vi "Lire un segment MODBUS EPC.vi"(0 "Port COM":refnum<visa-resource-name>, 1 "No prog":u8 caption="Numéro de programme", 2 "Adresse régulateur":u8, 3 "Numéro de segment":u8, 4 "données générales":u16[](array[numeric]), 5 "error in (no error)":errorcluster caption="entrée d'erreur (pas d'erreur)") -> (6 "Programmation Segment":T1(array[cluster]), 7 "Fin de programme":bool, 8 "error out":errorcluster caption="entrée d'erreur (pas d'erreur)")   [LabVIEW 2022 SP3]
uses:
  Variables globales/Variables glob EUROTHERM.vi
panel:
  out "Data 2 (U16)":u16[][](array[numeric])
  # "unités rampe"
  # "unités palier"
  # "nb cycles"
  # "type fin"
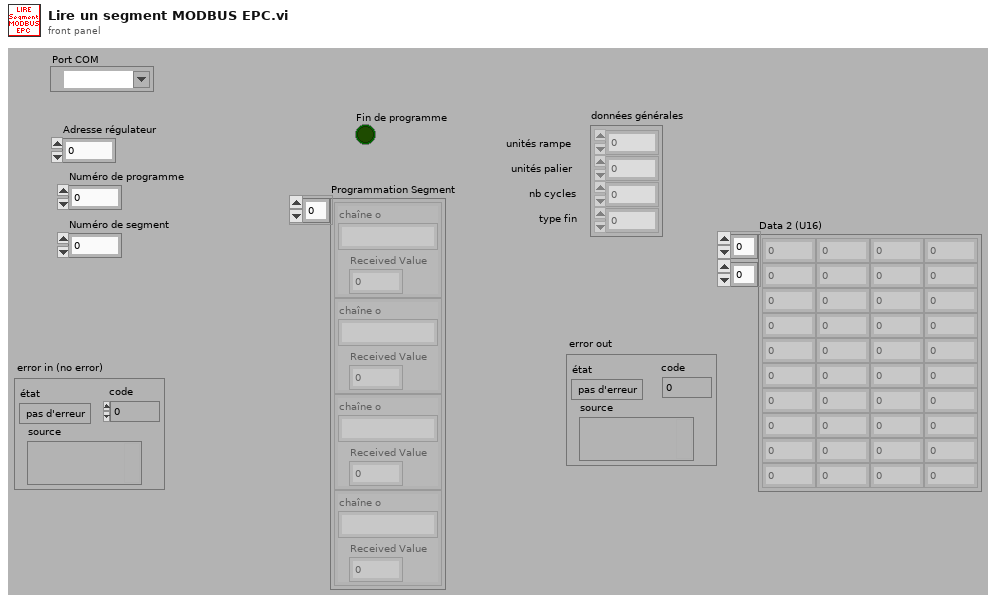
[diagram p1: front panel]
types:
  T1 = cluster{"chaîne o":string, "Received Value":dbl}[]
  T2 = typedef "Semaphore RefNum" = refnum<k1>
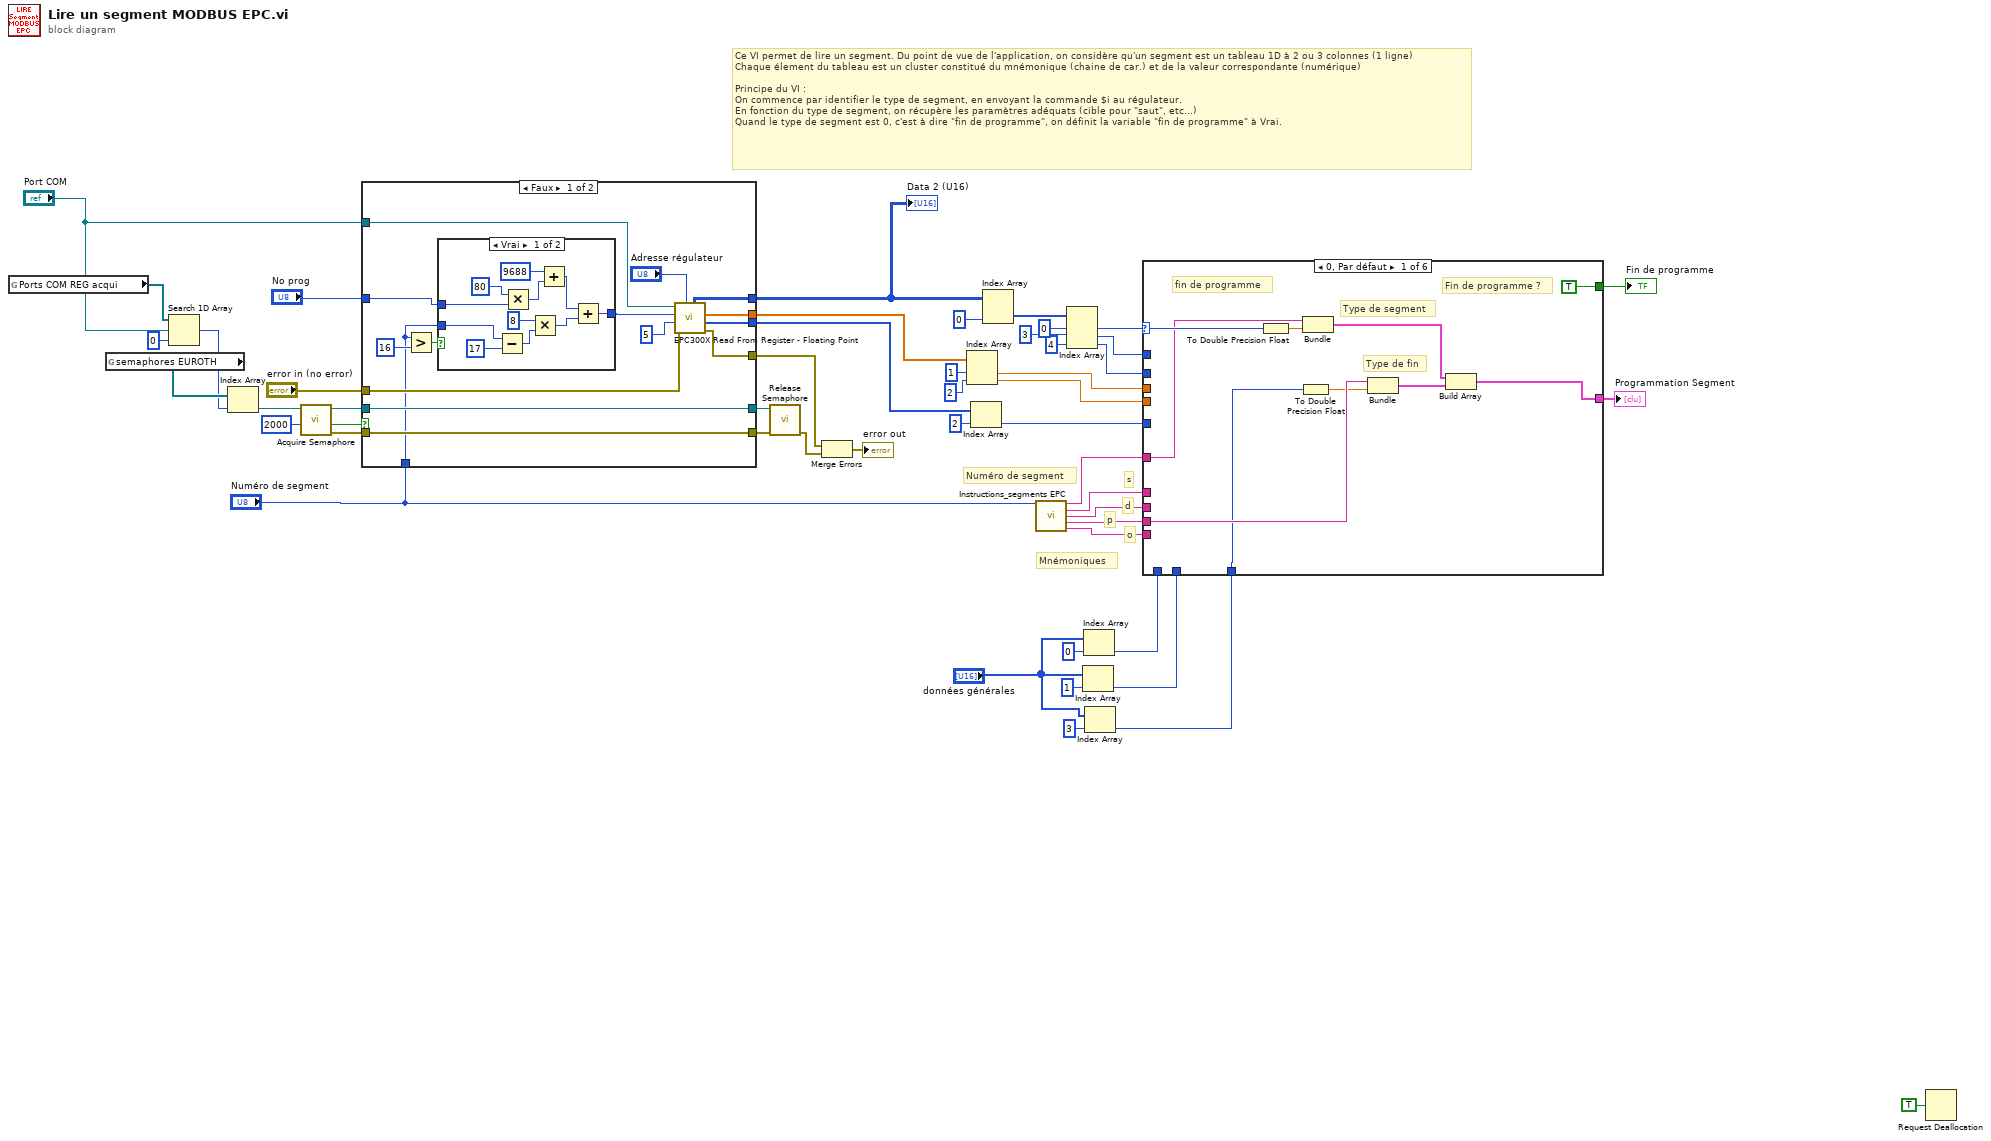
[diagram p0: block diagram]
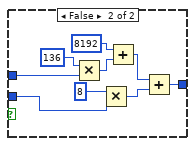
[diagram p2: hidden frame]
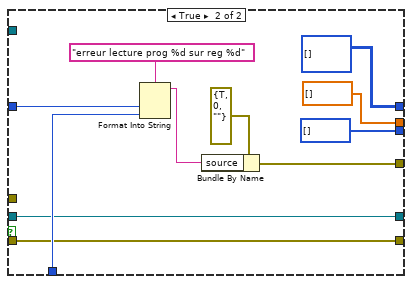
[diagram p3: hidden frame]
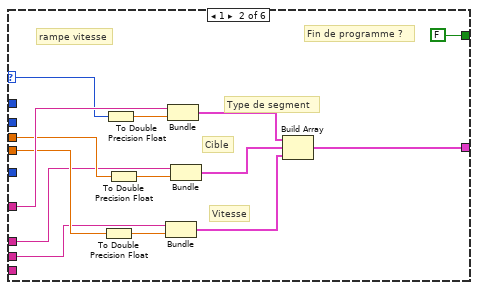
[diagram p4: hidden frame]
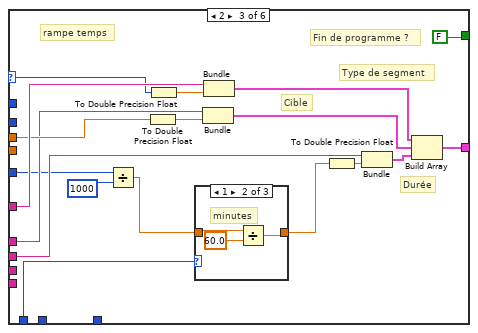
[diagram p5: hidden frame]
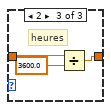
[diagram p7: hidden frame]
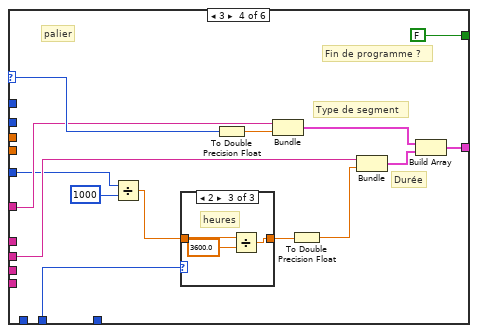
[diagram p8: hidden frame]
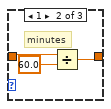
[diagram p10: hidden frame]
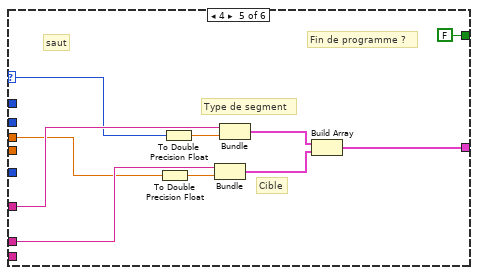
[diagram p11: hidden frame]
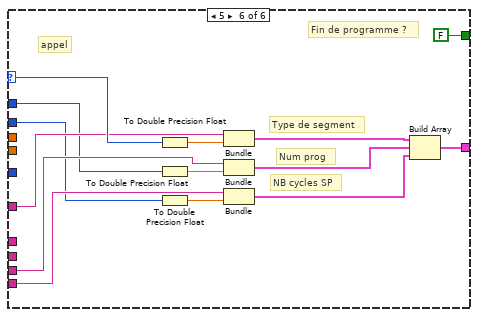
[diagram p12: hidden frame]
diagram:
  # "o"
  # "p"
  # "d"
  # "s"
  # "Ce VI permet de lire un segment. Du point de vue de l'application, on considère qu'un segment est un tableau 1D à 2 ou 3 colonnes (1 ligne)\nChaque élement du tableau est un cluster constitué du mnémonique (chaine de car.) et de la valeur correspondante (numérique)\n\nPrincipe du VI : \nOn commence par identifier le type de segment, en envoyant la commande $i au régulateur.\nEn fonction du type de segment, on récupère les paramètres adéquats (cible pour \"saut\", etc...)\nQuand le type de segment est 0, c'est à dire \"fin de programme\", on définit la variable \"fin de programme\" à Vrai."
  # "Mnémoniques"
  # "Numéro de segment"
  n1 = global read "Variables glob EUROTHERM.vi" "Ports COM REG acqui"() -> (w15:refnum<visa-resource-name>[])
  n2 = global read "Variables glob EUROTHERM.vi" "semaphores EUROTH"() -> (w12:T2[])
  n3 = Search 1D Array(1D array=w15, element="Port COM", start index (0)=0 ("indice de départ (0)")) -> (index of element=w10:i32)
  n4 = Index Array(array=w12, index=w10) -> (element=w13:T2)
  n5 = call <vilib>:"Acquire Semaphore.vi"("ms timeout (-1)"=2000, "semaphore"=w13) -> ("error out"=w7:errorcluster, "timed out"=w9:bool, "semaphore out"=w8:T2)  [unwired: 3 in]
  n6 = case shown="Faux" w9 {
    tunnel: "error in (no error)" -> [w63 _]
    tunnel: [w62 u16[][] [] ("Data 2 (U16)")] -> w34
    tunnel: [w61 sgl[] [] ("Data (SGL)")] -> w33
    tunnel: [w60 u32[] [] ("Data (ms)")] -> w32
    tunnel: [w59 w91] -> w4
    tunnel: "Port COM" -> [w58 _]
    tunnel: "Numéro de segment" -> [w53 w94]
    tunnel: w8 -> [w57 w90]
    tunnel: w7 -> [w56 w89]
    tunnel: [w57 w90] -> w6
    tunnel: [w56 w89] -> w3
    tunnel: "No prog" -> [w52 w95]
    frame False {
      n7 = Greater?(x=w53, y=u16 16) -> (0:w54:bool)
      n8 = case shown="Vrai" w54 {
        tunnel: w53 -> [w68 w78]
        tunnel: w52 -> [w67 w79]
        tunnel: [w66 w77] -> w51
        frame True {
          n9 = Subtract(x=w68, y=u16 17) -> (x-y=w69:u16)
          n10 = Multiply(x=u16 80, y=w67) -> (x*y=w73:u16)
          n11 = Multiply(x=u16 8, y=w69) -> (x*y=w75:u16)
          n12 = Add(x=u16 9688, y=w73) -> (x+y=w71:u16)
          n13 = Add(x=w71, y=w75) -> (x+y=w66:u16)
        }
        frame False {
          n14 = Multiply(x=u16 136, y=w79) -> (x*y=w82:u16)
          n15 = Multiply(x=u16 8, y=w78) -> (x*y=w84:u16)
          n16 = Add(x=u16 8192, y=w82) -> (x+y=w80:u16)
          n17 = Add(x=w80, y=w84) -> (x+y=w77:u16)
        }
      }
      n18 = call "EPC300X Read From Register - Floating Point.vi"("Unit Address (1)"="Adresse régulateur", "error in (no error)"=w63, "Num Of Reg (1)"=u16 5, "Register Address (0)"=w51, "VISA session"=w58) -> ("error out"=w59:errorcluster, "Data (ms)"=w60:u32[], "Data (SGL)"=w61:sgl[], "Data 2 (U16)"=w62:u16[][])  [unwired: 1 in, 2 out]
    }
    frame True {
      n19 = Format Into String(format string="erreur lecture prog %d sur reg %d" ("chaîne de format"), w95, w94) -> (resulting string=w92:string)  [unwired: 2 in, 1 out]
      n20 = Bundle By Name(cluster=errorcluster {"status"=TRUE, "code"=0, "source"=""} ("error out"), "source"=w92) -> (w91:errorcluster)
    }
  }
  "Data 2 (U16)" <- w34
  n21 = call <vilib>:"Release Semaphore.vi"("error in (no error)"=w3, "semaphore"=w6) -> ("error out"=w1:errorcluster)  [unwired: 4 in, 1 out]
  n22 = Merge Errors(w4, w1) -> (→"error out":errorcluster)
  n23 = Index Array(array=w33, index #1=1 ("indice"), index #2=2 ("indice")) -> (element #1=w37:sgl, element #2=w36:sgl)
  n24 = Index Array(array=w32, index=2 ("indice")) -> (element=w35:u32)
  n25 = Index Array(array=w34, index (col)=0 ("indice (ligne)")) -> (element=w43:u16[])  [unwired: 1 in]
  n26 = call "Instructions_segments EPC.vi"("Numéro de segment"="Numéro de segment") -> ("chaîne $"=w31:string, "chaîne s"=w29:string, "chaîne d"=w30:string, "chaîne p"=w28:string, "chaîne o"=w27:string)  [unwired: 10 in]
  n27 = Index Array(array=w43, index #1=0 ("indice"), index #2=3 ("indice"), index #3=4 ("indice")) -> (element #1=w42:u16, element #2=w39:u16, element #3=w38:u16)
  n28 = Index Array(array="données générales", index=1 ("indice")) -> (element=w21:u16)
  n29 = Index Array(array="données générales", index=0 ("indice")) -> (element=w18:u16)
  n30 = Index Array(array="données générales", index=3 ("indice")) -> (element=w22:u16)
  n31 = case shown="0, Par défaut" w42 {
    selector: w42 -> [w103 w116 w135 w155 w170 w186]
    tunnel: w39 -> [_ _ _ _ _ w182]
    tunnel: w38 -> [_ _ _ _ _ w181]
    tunnel: w37 -> [_ w114 w131 _ w169 _]
    tunnel: w36 -> [_ w112 _ _ _ _]
    tunnel: w35 -> [_ _ w124 w152 _ _]
    tunnel: w31 -> [w102 w117 w136 w154 w172 w185]
    tunnel: w30 -> [_ w110 w128 w153 _ _]
    tunnel: w29 -> [_ w111 w130 _ w171 _]
    tunnel: w28 -> [w101 _ _ _ _ w184]
    tunnel: w27 -> [_ _ _ _ _ w183]
    tunnel: [w100 w108 w126 w151 w168 w177] -> w26
    tunnel: [TRUE FALSE FALSE FALSE FALSE FALSE] -> w25
    tunnel: w22 -> [w97 _ _ _ _ _]
    tunnel: w21 -> [_ _ _ w149 _ _]
    tunnel: w18 -> [_ _ w122 _ _ _]
    frame 0, Default {
      # "Type de fin"
      # "Type de segment"
      # "Fin de programme ?"
      # "fin de programme"
      n32 = To Double Precision Float(number=w103) -> (double precision float=w105:dbl)
      n33 = To Double Precision Float(number=w97) -> (double precision float=w99:dbl)
      n34 = Bundle("chaîne $"=w102, w105) -> (w104:cluster{"chaîne $":string, dbl})  [unwired: 1 in]
      n35 = Bundle("chaîne p"=w101, w99) -> (w98:cluster{"chaîne p":string, dbl})  [unwired: 1 in]
      n36 = Build Array(w104, w98) -> (w100:cluster{"chaîne p":string, dbl}[])
    }
    frame 1 {
      # "Fin de programme ?"
      # "Vitesse"
      # "Cible"
      # "Type de segment"
      # "rampe vitesse"
      n37 = To Double Precision Float(number=w112) -> (double precision float=w118:dbl)
      n38 = To Double Precision Float(number=w116) -> (double precision float=w120:dbl)
      n39 = To Double Precision Float(number=w114) -> (double precision float=w119:dbl)
      n40 = Bundle("chaîne d"=w110, w118) -> (w109:cluster{"chaîne d":string, dbl})  [unwired: 1 in]
      n41 = Bundle("chaîne $"=w117, w120) -> (w115:cluster{"chaîne $":string, dbl})  [unwired: 1 in]
      n42 = Bundle("chaîne s"=w111, w119) -> (w113:cluster{"chaîne s":string, dbl})  [unwired: 1 in]
      n43 = Build Array(w115, w113, w109) -> (w108:cluster{"chaîne d":string, dbl}[])
    }
    frame 2 {
      # "Durée"
      # "Cible"
      # "Type de segment"
      # "Fin de programme ?"
      # "rampe temps"
      n44 = Divide(x=w124, y=u32 1000) -> (x/y=w125:dbl)
      n45 = To Double Precision Float(number=w131) -> (double precision float=w134:dbl)
      n46 = To Double Precision Float(number=w135) -> (double precision float=w137:dbl)
      n47 = case shown="1" w122 {
        tunnel: w125 -> [w139 w142 w145]
        tunnel: [w139 w140 w143] -> w123
        frame 0, Default {
          # "secondes"
        }
        frame 1 {
          # "minutes"
          n48 = Divide(x=w142, y=60.0) -> (x/y=w140:dbl)
        }
        frame 2 {
          # "heures"
          n49 = Divide(x=w145, y=3600.0) -> (x/y=w143:dbl)
        }
      }
      n50 = Bundle("chaîne s"=w130, w134) -> (w129:cluster{"chaîne s":string, dbl})  [unwired: 1 in]
      n51 = Bundle("chaîne $"=w136, w137) -> (w132:cluster{"chaîne $":string, dbl})  [unwired: 1 in]
      n52 = To Double Precision Float(number=w123) -> (double precision float=w133:dbl)
      n53 = Bundle("chaîne d"=w128, w133) -> (w127:cluster{"chaîne d":string, dbl})  [unwired: 1 in]
      n54 = Build Array(w132, w129, w127) -> (w126:cluster{"chaîne d":string, dbl}[])
    }
    frame 3 {
      # "Fin de programme ?"
      # "Durée"
      # "Type de segment"
      # "palier"
      n55 = Divide(x=w152, y=u32 1000) -> (x/y=w148:dbl)
      n56 = case shown="2" w149 {
        tunnel: w148 -> [w160 w163 w166]
        tunnel: [w160 w161 w164] -> w147
        frame 0, Default {
          # "secondes"
        }
        frame 1 {
          # "minutes"
          n57 = Divide(x=w163, y=60.0) -> (x/y=w161:dbl)
        }
        frame 2 {
          # "heures"
          n58 = Divide(x=w166, y=3600.0) -> (x/y=w164:dbl)
        }
      }
      n59 = To Double Precision Float(number=w155) -> (double precision float=w159:dbl)
      n60 = Bundle("chaîne $"=w154, w159) -> (w156:cluster{"chaîne $":string, dbl})  [unwired: 1 in]
      n61 = To Double Precision Float(number=w147) -> (double precision float=w158:dbl)
      n62 = Bundle("chaîne d"=w153, w158) -> (w157:cluster{"chaîne d":string, dbl})  [unwired: 1 in]
      n63 = Build Array(w156, w157) -> (w151:cluster{"chaîne d":string, dbl}[])
    }
    frame 4 {
      # "Fin de programme ?"
      # "Cible"
      # "Type de segment"
      # "saut"
      n64 = To Double Precision Float(number=w169) -> (double precision float=w175:dbl)
      n65 = To Double Precision Float(number=w170) -> (double precision float=w176:dbl)
      n66 = Bundle("chaîne s"=w171, w175) -> (w174:cluster{"chaîne s":string, dbl})  [unwired: 1 in]
      n67 = Bundle("chaîne $"=w172, w176) -> (w173:cluster{"chaîne $":string, dbl})  [unwired: 1 in]
      n68 = Build Array(w173, w174) -> (w168:cluster{"chaîne s":string, dbl}[])
    }
    frame 5 {
      # "NB cycles SP"
      # "Num prog"
      # "Type de segment"
      # "Fin de programme ?"
      # "appel"
      n69 = To Double Precision Float(number=w186) -> (double precision float=w189:dbl)
      n70 = To Double Precision Float(number=w182) -> (double precision float=w188:dbl)
      n71 = To Double Precision Float(number=w181) -> (double precision float=w187:dbl)
      n72 = Bundle("chaîne $"=w185, w189) -> (w180:cluster{"chaîne $":string, dbl})  [unwired: 1 in]
      n73 = Bundle("chaîne p"=w184, w188) -> (w179:cluster{"chaîne p":string, dbl})  [unwired: 1 in]
      n74 = Bundle("chaîne o"=w183, w187) -> (w178:cluster{"chaîne o":string, dbl})  [unwired: 1 in]
      n75 = Build Array(w180, w179, w178) -> (w177:cluster{"chaîne o":string, dbl}[])
    }
  }
  "Fin de programme" <- w25
  "Programmation Segment" <- w26
  n76 = Request Deallocation(TRUE ("flag")) -> ()
